vi "SPI.vi"() -> ()   [LabVIEW 2012]
uses:
  USB2UARTSPIIICDLL.dll
panel:
  in  "SPI接收长度":dbl
  in  "SPI发送长度":dbl
  in  "数组 2":i8[](array[numeric]) format="%x"
  out "CloseUsb函数返回值":dbl
  in  "数组":i8[](array[numeric]) format="%x"
  out "SPISendAndRcvData0函数返回值":dbl
  out "ConfigSPIParam函数返回值":dbl
  in  "SPI速率":dbl
  in  "开始测试按钮":bool
  out "OpenUsb函数返回值":dbl
  in  "UsbIndex":dbl
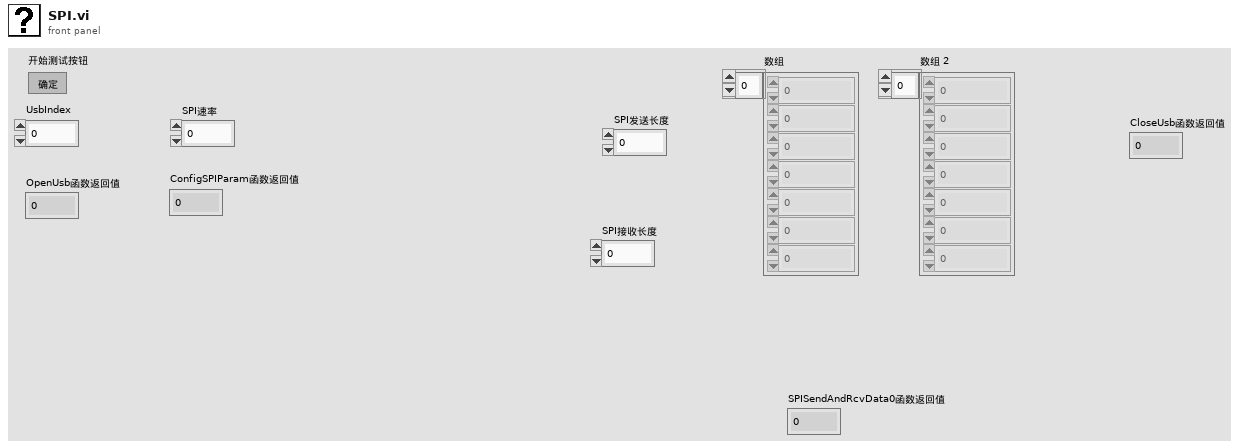
[diagram p1: front panel]
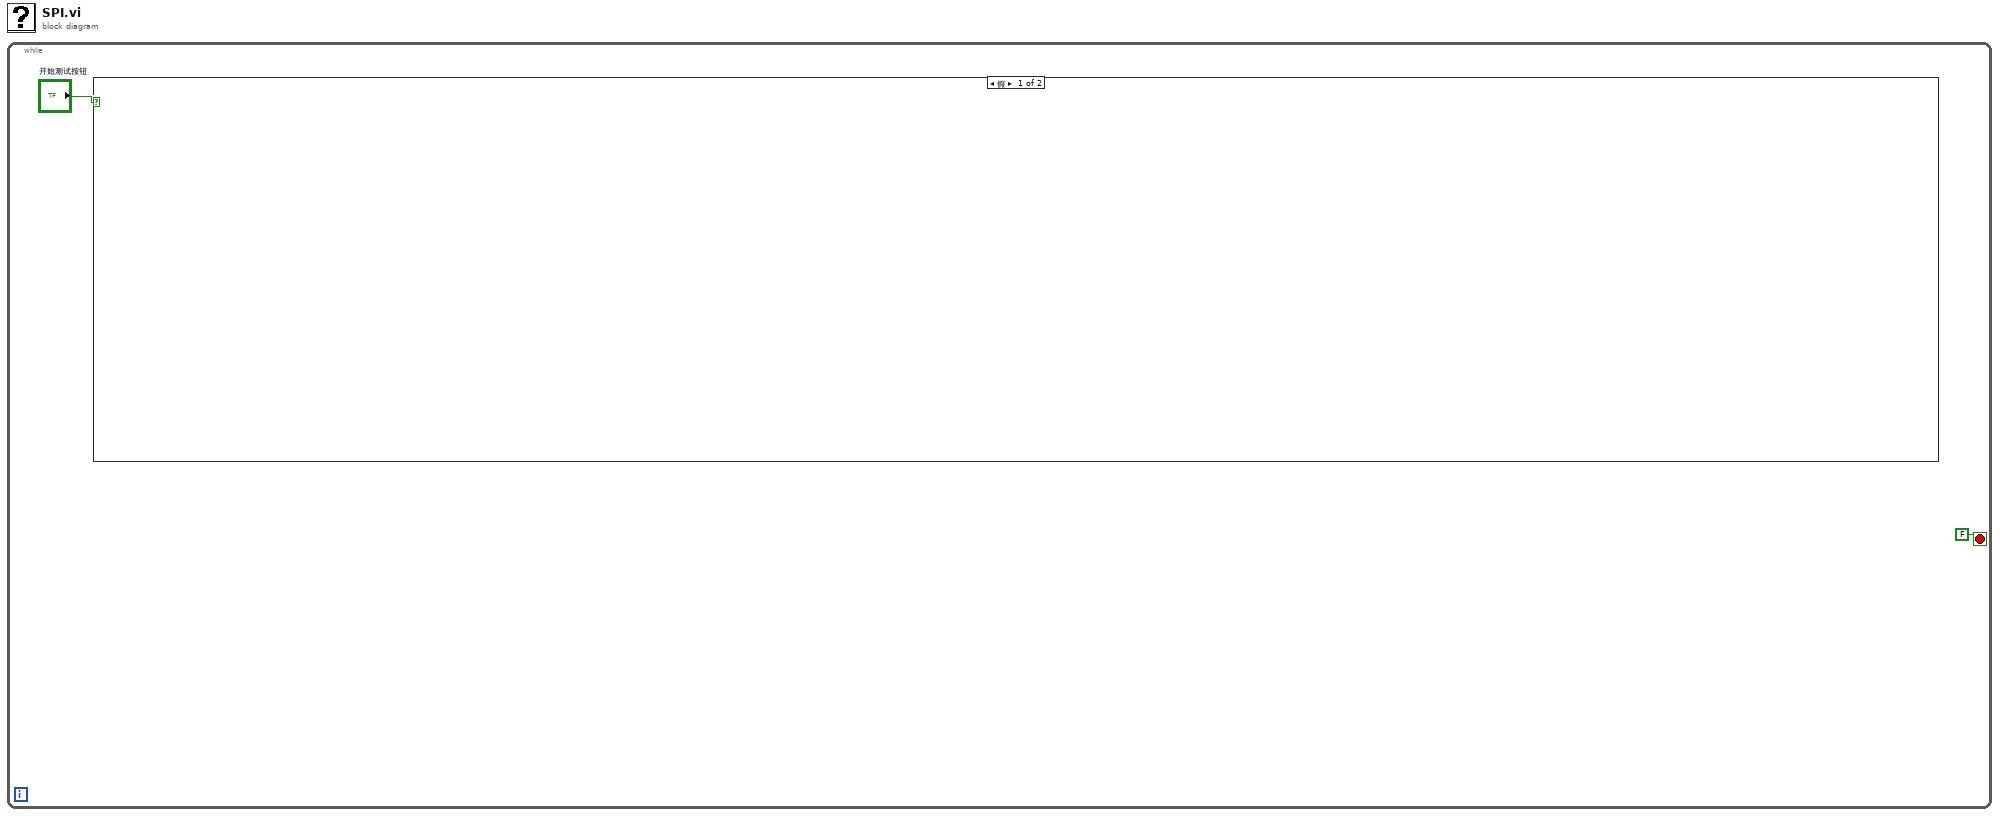
[diagram p0: block diagram]
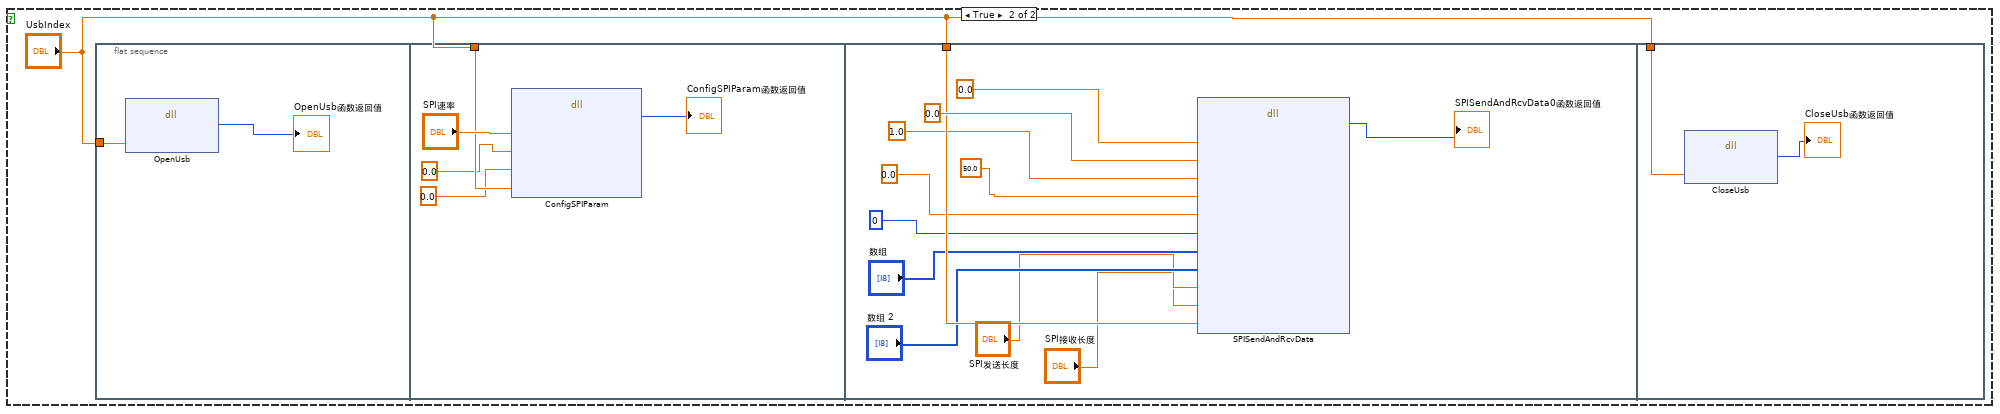
[diagram p2: hidden frame]
diagram:
  n1 = while {
    stop <- FALSE stop-if-true
    n2 = case shown="假" "开始测试按钮" {
      frame False {
      }
      frame True {
        n3 = flat-sequence "平铺式顺序结构" {
          tunnel: "UsbIndex" -> [w5]
          tunnel: "UsbIndex" -> [w9]
          tunnel: "UsbIndex" -> [w20]
          tunnel: "UsbIndex" -> [w24]
          frame #0 {
            n4 = dll-call lib="F:/work/USB2SPIUARTIIC/103/SW/Labview/SPI/USB2UARTSPIIICDLL.dll" fn="OpenUsb"("UsbIndex"=w5) -> ("返回类型"=→"OpenUsb函数返回值":i32)  [unwired: 4 in, 2 out]
          }
          frame #1 {
            n5 = dll-call lib="F:/work/USB2SPIUARTIIC/103/SW/Labview/SPI/USB2UARTSPIIICDLL.dll" fn="ConfigSPIParam"("rate"="SPI速率", "fistBit"=0.0 ("strartBit"), "subMode"=0.0 ("strartBit"), "UsbIndex"=w9) -> ("返回类型"=→"ConfigSPIParam函数返回值":i32)  [unwired: 7 in, 2 out]
          }
          frame #2 {
            n6 = dll-call lib="F:/work/USB2SPIUARTIIC/103/SW/Labview/SPI/USB2UARTSPIIICDLL.dll" fn="SPISendAndRcvData"("CSshelect"=0.0 ("strartBit"), "startCS"=0.0 ("strartBit"), "endCS"=1.0 ("strartBit"), "CSdelay"=50.0 ("strartBit"), "duplex"=0.0 ("strartBit"), "dummy"=i16 0 ("strartBit"), "sendBuf"="数组", "rcvBuf"="数组 2", "slen"="SPI发送长度", "rlen"="SPI接收长度", "UsbIndex"=w20) -> ("返回类型"=→"SPISendAndRcvData0函数返回值":i32)  [unwired: 14 in, 2 out]
          }
          frame #3 {
            n7 = dll-call lib="F:/work/USB2SPIUARTIIC/103/SW/Labview/SPI/USB2UARTSPIIICDLL.dll" fn="CloseUsb"("UsbIndex"=w24) -> ("返回类型"=→"CloseUsb函数返回值":i32)  [unwired: 4 in, 2 out]
          }
        }
      }
    }
  }
